vi "write_then_read.vi"() -> ()   [LabVIEW 2016]
panel:
  in  "Type something here":string
  out "File content":string
  in  "Path":path
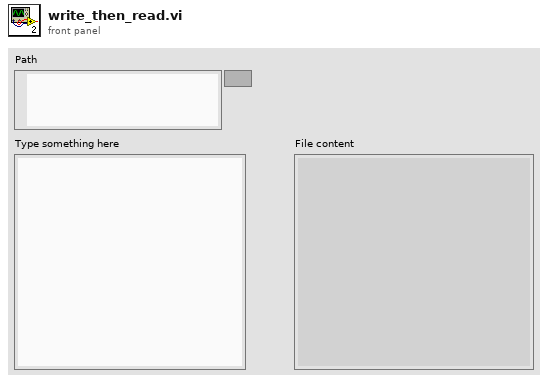
[diagram p1: front panel]
types:
  T1 = enum16{"open", "replace", "create", "open or create", "replace or create", "replace or create with confirmation"}
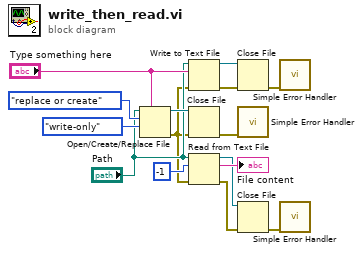
[diagram p0: block diagram]
diagram:
  n1 = Open/Create/Replace File(file path (use dialog)="Path", prompt="Type something here", operation (0:open)=T1."replace or create", access (0:read/write)=enum16{"read/write", "read-only", "write-only"}."write-only") -> (refnum out=w13:refnum<file>, error out=w1:errorcluster)  [unwired: 2 in, 1 out]
  n2 = Write to Text File(file (use dialog)="Path", text="Type something here", error in=w1) -> (refnum out=w3:refnum<file>, error out=w2:errorcluster)  [unwired: 1 in, 1 out]
  n3 = Close File(refnum=w13, error in=w1) -> (error out=w12:errorcluster)  [unwired: 1 out]
  n4 = Read from Text File(file (use dialog)="Path", count=-1, error in=w1) -> (refnum out=w9:refnum<file>, text=→"File content":string, error out=w8:errorcluster)  [unwired: 1 in, 1 out]
  n5 = Close File(refnum=w3, error in=w2) -> (error out=w4:errorcluster)  [unwired: 1 out]
  n6 = call <vilib>:"Simple Error Handler.vi"("error in (no error)"=w12) -> ()  [unwired: 4 in, 5 out]
  n7 = Close File(refnum=w9, error in=w8) -> (error out=w7:errorcluster)  [unwired: 1 out]
  n8 = call <vilib>:"Simple Error Handler.vi"("error in (no error)"=w4) -> ()  [unwired: 4 in, 5 out]
  n9 = call <vilib>:"Simple Error Handler.vi"("error in (no error)"=w7) -> ()  [unwired: 4 in, 5 out]
